vi "ZM-CU-log.vi"(8 "error in":errorcluster, 11 "message":string) -> (0 "error out":errorcluster)   [LabVIEW 2020, in "ZM-CU-common_utilities.lvlib"]
doc: "The project's local error log: appends one line, <ISO UTC timestamp><tab><message>, to output/ZM-error_log.txt in the project folder, creating the folder if missing. It logs regardless of error in."
uses:
  ZM-CU-common_utilities.lvlib
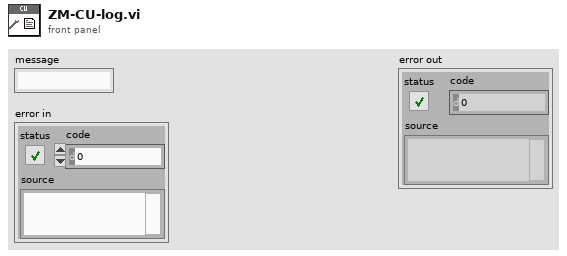
[diagram p1: front panel]
types:
  T1 = enum16{"open", "replace", "create", "open or create", "replace or create", "replace or create with confirmation"}
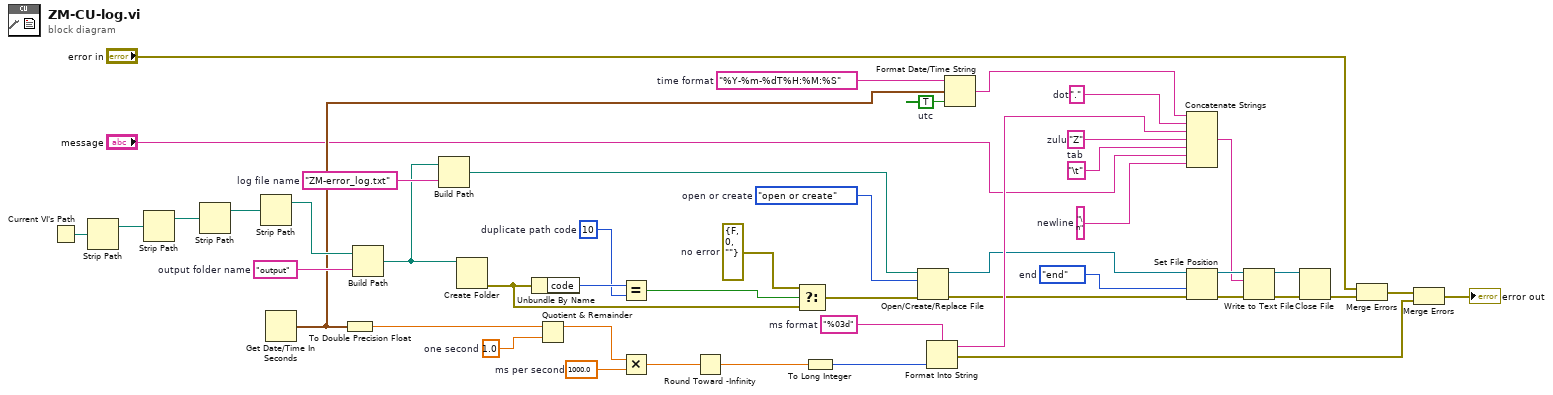
[diagram p0: block diagram]
diagram:
  w12 = enum16{"start", "end", "current"}."end"  # end
  w15 = T1."open or create"  # open or create
  w19 = errorcluster {"status"=FALSE, "code"=0, "source"=""}  # no error
  w20 = 10  # duplicate path code
  w23 = "\n"  # newline
  w25 = "\t"  # tab
  w26 = "Z"  # zulu
  w28 = "."  # dot
  w31 = "%03d"  # ms format
  w34 = 1000.0  # ms per second
  w36 = 1.0  # one second
  w39 = TRUE  # utc
  w40 = "%Y-%m-%dT%H:%M:%S"  # time format
  w41 = "ZM-error_log.txt"  # log file name
  w42 = "output"  # output folder name
  n1 = Current VI's Path() -> (path=w47:path)
  n2 = Strip Path(path=w47) -> (stripped path=w46:path)  [unwired: 1 out]
  n3 = Strip Path(path=w46) -> (stripped path=w45:path)  [unwired: 1 out]
  n4 = Strip Path(path=w45) -> (stripped path=w44:path)  [unwired: 1 out]
  n5 = Strip Path(path=w44) -> (stripped path=w43:path)  [unwired: 1 out]
  n6 = Get Date/Time In Seconds() -> (seconds since 1Jan1904=w38:timestamp)
  n7 = To Double Precision Float(number=w38) -> (double precision float=w37:dbl)
  n8 = Build Path(base path=w43, name or relative path=w42) -> (appended path=w22:path)
  n9 = Build Path(base path=w22, name or relative path=w41) -> (appended path=w16:path)
  n10 = Create Folder(path (use dialog)=w22) -> (error out=w17:errorcluster)  [unwired: 2 in, 2 out]
  n11 = Unbundle By Name(w17) -> ("code"=w21:i32)
  n12 = Quotient & Remainder(x=w37, y=w36) -> (x-y*floor(x/y)=w35:dbl)  [unwired: 1 out]
  n13 = Equal?(x=w21, y=w20) -> (x = y?=w18:bool)
  n14 = Multiply(x=w35, y=w34) -> (x*y=w33:dbl)
  n15 = Round Toward -Infinity(1:w33) -> (0:w32:dbl)
  n16 = Select(t=w19, s=w18, f=w17) -> (s? t:f=w14:errorcluster)
  n17 = To Long Integer(number=w32) -> (32bit integer=w30:i32)
  n18 = Open/Create/Replace File(file path (use dialog)=w16, error in=w14, operation (0:open)=w15) -> (refnum out=w13:refnum<file>, error out=w11:errorcluster)  [unwired: 3 in, 1 out]
  n19 = Format Into String(format string=w31, w30) -> (resulting string=w27:string, error out=w2:errorcluster)  [unwired: 2 in]
  n20 = Format Date/Time String(time format string (%c)=w40, seconds (now)=w38, UTC format=w39) -> (date/time string=w29:string)
  n21 = Concatenate Strings(w29, w28, w27, w26, w25, "message", w23) -> (w9:string)
  n22 = Set File Position(refnum=w13, from (0:start)=w12, error in=w11) -> (refnum out=w10:refnum<file>, error out=w8:errorcluster)  [unwired: 1 in]
  n23 = Write to Text File(file (use dialog)=w10, text=w9, error in=w8) -> (refnum out=w7:refnum<file>, error out=w6:errorcluster)  [unwired: 1 in, 1 out]
  n24 = Close File(refnum=w7, error in=w6) -> (error out=w4:errorcluster)  [unwired: 1 out]
  n25 = Merge Errors("error in", w4) -> (w3:errorcluster)
  n26 = Merge Errors(w3, w2) -> (→"error out":errorcluster)
